vi "测试数据保存.vi"(7 "文件名称前缀":string, 8 "错误输入（无错误）":errorcluster, 10 "数据":dbl[][](array[numeric]), 11 "start path":path=path "D:/Data") -> (0 "错误输出":errorcluster)   [LabVIEW 2020]
uses:
  <vilib>/Utility/file.llb/Write Delimited Spreadsheet (DBL).vi
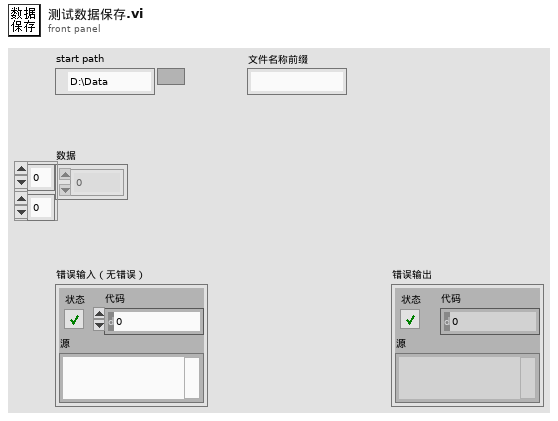
[diagram p1: front panel]
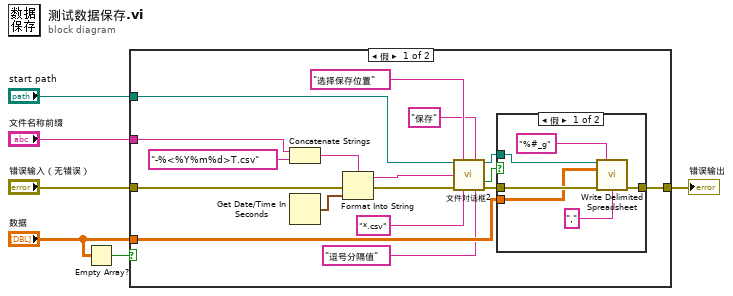
[diagram p0: block diagram]
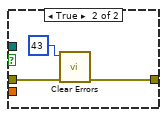
[diagram p2: hidden frame]
diagram:
  n1 = Empty Array?(array="数据") -> (empty?=w5:bool)
  n2 = case shown="假" w5 {
    tunnel: "数据" -> [w23 _]
    tunnel: [w11 w33] -> w3
    tunnel: "错误输入（无错误）" -> [w10 w33]
    tunnel: "文件名称前缀" -> [w8 _]
    tunnel: "start path" -> [w7 _]
    frame False {
      n3 = Concatenate Strings(w8, "-%<%Y%m%d>T.csv" ("格式字符串")) -> (w9:string)
      n4 = Get Date/Time In Seconds() -> (seconds since 1Jan1904=w13:timestamp)
      n5 = Format Into String(format string=w9, error in=w10, w13) -> (resulting string=w15:string, error out=w14:errorcluster)  [unwired: 1 in]
      n6 = call "文件对话框2"("start path"=w7, "prompt"="选择保存位置", "button label"="保存", "default name"=w15, "error in"=w14, "pattern (all files)"="*.csv", "pattern label"="逗号分隔值") -> ("selected path"=w21:path, "cancelled"=w22:bool, "error out"=w19:errorcluster)  [unwired: 5 in, 1 out]
      n7 = case shown="假" w22 {
        tunnel: w19 -> [w29 w32]
        tunnel: [w28 w31] -> w11
        tunnel: w21 -> [w27 _]
        tunnel: w23 -> [w26 _]
        frame False {
          n8 = call-poly <vilib>:"Write Delimited Spreadsheet.vi"("file path (dialog if empty)"=w27, "format (%.3f)"="%#_g", "2D data"=w26, "error in (no error)"=w29, "delimiter (\\t)"="," ("delimiter (\\t)")) -> ("error out"=w28:errorcluster)  [unwired: 9 in, 1 out]
        }
        frame True {
          n9 = call <vilib>:"Clear Errors.vi"("error in (no error)"=w32, "specific error code to clear (0: all)"=43) -> ("error out"=w31:errorcluster)  [unwired: 4 in, 1 out]
        }
      }
    }
    frame True {
    }
  }
  "错误输出" <- w3
